vi "RemoteVI Stop.vi"(0 "port":u16=8088, 11 "error in":errorcluster) -> (15 "error out":errorcluster)   [LabVIEW 2020, in "RemoteVI.lvlib"]
doc: "Stops the server that RemoteVI Start.vi launched on port: obtains the notifier RemoteVI:<port> without creating it, sends a notification and releases it, then waits up to 2 s for ..\\Server\\RemoteVI Server Loop.vi to go idle, so the port is free when this VI returns. No server on that port is not an error. Runs even when error in carries an error, and merges its own errors after it."
uses:
  RemoteVI.lvlib
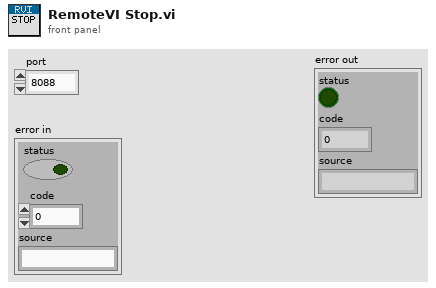
[diagram p1: front panel]
types:
  T1 = enum32{"Bad", "Idle", "Run top level", "Running"}
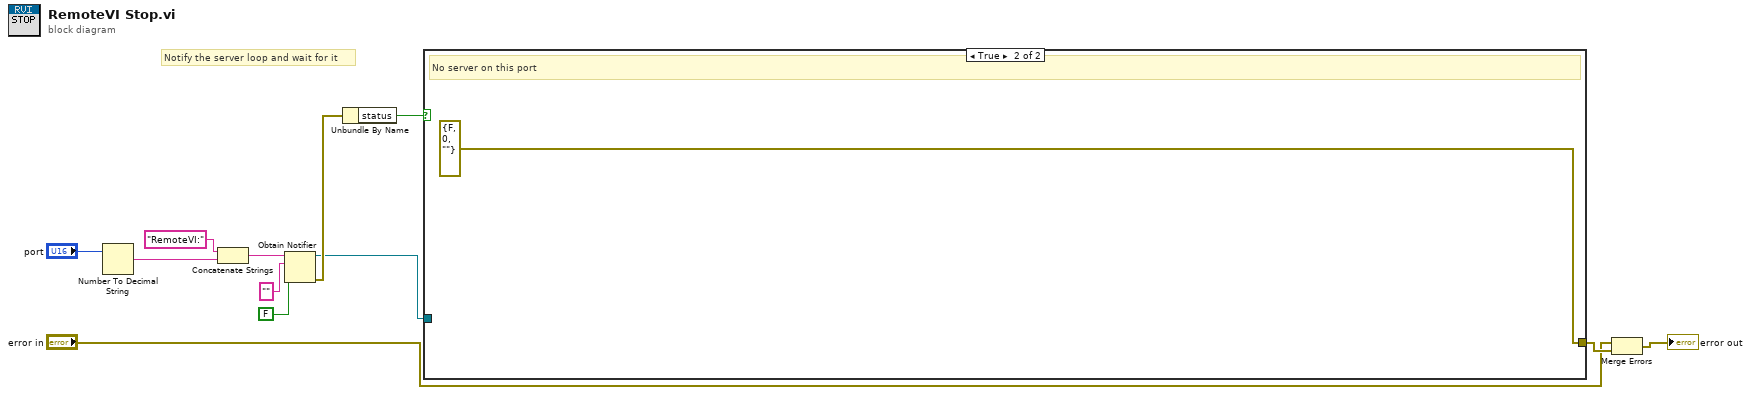
[diagram p0: block diagram]
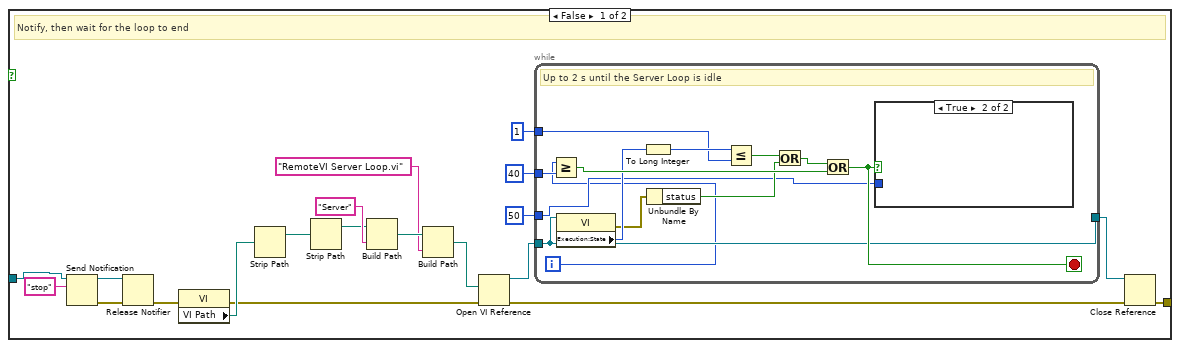
[diagram p2: hidden frame]
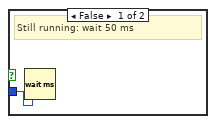
[diagram p3: hidden frame]
diagram:
  # "Notify the server loop and wait for it"
  n1 = Number To Decimal String(number="port") -> (decimal integer string=w4:string)  [unwired: 1 in]
  n2 = Concatenate Strings("RemoteVI:", w4) -> (w5:string)
  n3 = Obtain Notifier(name (unnamed)=w5, notification data type="", create if not found? (T)=FALSE) -> (notifier out=w8:refnum<notifier>, error out=w9:errorcluster)  [unwired: 1 in, 1 out]
  n4 = Unbundle By Name(w9) -> ("status"=w10:bool)
  n5 = case shown="True" w10 {
    tunnel: [w32 errorcluster {"status"=FALSE, "code"=0, "source"=""}] -> w11
    tunnel: w8 -> [w13 _]
    frame False {
      # "Notify, then wait for the loop to end"
      n6 = Send Notification(notification="stop", notifier=w13) -> (notifier out=w15:refnum<notifier>, error out=w16:errorcluster)  [unwired: 1 in]
      n7 = Release Notifier(notifier=w15, error in (no error)=w16) -> (error out=w17:errorcluster)  [unwired: 1 in, 2 out]
      n8 = property class="VI"(error in=w17) -> (error out=w18:errorcluster, "VI Path"=w19:path)  [unwired: 1 in, 1 out]
      n9 = Strip Path(path=w19) -> (stripped path=w20:path)  [unwired: 1 out]
      n10 = Strip Path(path=w20) -> (stripped path=w21:path)  [unwired: 1 out]
      n11 = Build Path(base path=w21, name or relative path="Server") -> (appended path=w24:path)
      n12 = Build Path(base path=w24, name or relative path="RemoteVI Server Loop.vi") -> (appended path=w25:path)
      n13 = Open VI Reference(vi path=w25, error in (no error)=w18) -> (vi reference=w26:refnum<vi>, error out=w27:errorcluster)  [unwired: 4 in]
      n14 = while {
        tunnel: 40 -> [w35]
        tunnel: 1 -> [w36]
        tunnel: 50 -> [w37]
        tunnel: w26 -> [w34]
        tunnel: [w34] -> w31
        i -> [w33]
        stop <- w45 stop-if-true
        # "Up to 2 s until the Server Loop is idle"
        n15 = Greater Or Equal?(x=w33, y=w35) -> (x >= y?=w43:bool)
        n16 = property class="VI"(reference=w34) -> (error out=w38:errorcluster, "Execution:State"=w39:T1)  [unwired: 1 in, 1 out]
        n17 = To Long Integer(number=w39) -> (32bit integer=w40:i32)
        n18 = Unbundle By Name(w38) -> ("status"=w42:bool)
        n19 = Less Or Equal?(x=w40, y=w36) -> (x <= y?=w41:bool)
        n20 = Or(x=w41, y=w42) -> (x .or. y?=w44:bool)
        n21 = Or(x=w44, y=w43) -> (x .or. y?=w45:bool)
        n22 = case shown="True" w45 {
          tunnel: w37 -> [w46 _]
          frame False {
            # "Still running: wait 50 ms"
            n23 = Wait (ms)(milliseconds to wait=w46) -> ()  [unwired: 1 out]
          }
          frame True {
          }
        }
      }
      n24 = Close Reference(reference=w31, error in (no error)=w27) -> (error out=w32:errorcluster)
    }
    frame True {
      # "No server on this port"
    }
  }
  n25 = Merge Errors("error in", w11) -> (→"error out":errorcluster)
